vi "Signal Table Anal.vi"(6 "error in (no error)":errorcluster caption="error in", 10 "Signal Table":string[][](table) caption="S Table", 11 "Signal Tag":string[](array[string])) -> (0 "MxRight":string[](array[string]), 1 "Assigned":string[](array[string]), 2 "RR":i32[](array[numeric]), 3 "AR":i32[](array[numeric]), 4 "error out":errorcluster, 5 "Direction":bool[](array[boolean]))   [LabVIEW 2018]
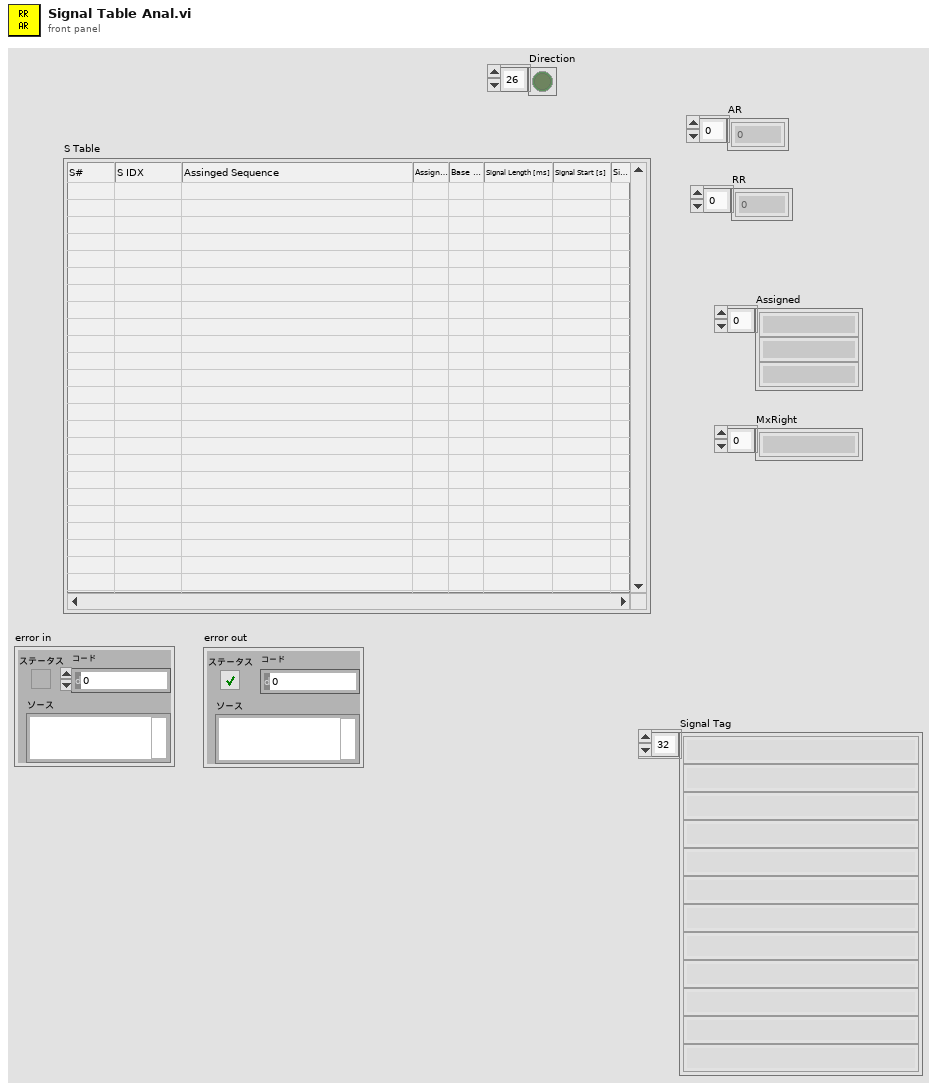
[diagram p1: front panel]
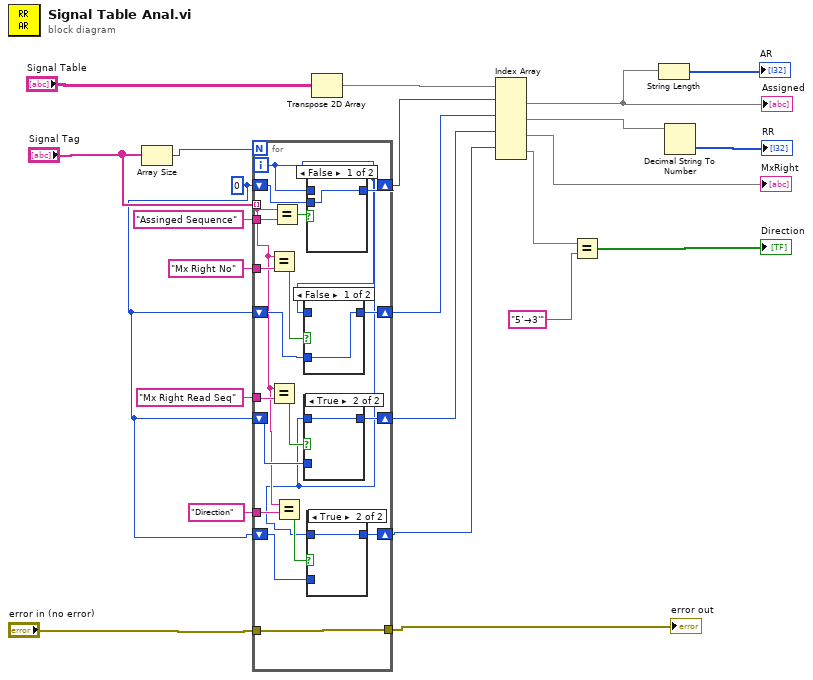
[diagram p0: block diagram]
diagram:
  w5 = 0
  n1 = Array Size(array="Signal Tag") -> (size(s)=w23:i32)
  n2 = for {
    N: w23 -> [_]
    tunnel: "Signal Tag" -> [w28] mode=indexing
    tunnel: "Assinged Sequence" ("グループ名入力") -> [w42]
    shift-right: [w40] -> w17
    shift-left: w5 -> [w41]
    tunnel: "Mx Right No" ("グループ名入力") -> [w36]
    shift-right: [w38] -> w16
    shift-left: w5 -> [w37]
    shift-right: [w32] -> w15
    shift-left: w5 -> [w31]
    tunnel: "Mx Right Read Seq" ("グループ名入力") -> [w33]
    tunnel: "error in (no error)" -> [w30]
    tunnel: [w30] -> w7
    tunnel: "Direction" ("グループ名入力") -> [w27]
    shift-right: [w25] -> w4
    shift-left: w5 -> [w26]
    i -> [w24]
    n3 = Equal?(x=w28, y=w36) -> (x = y?=w35:bool)
    n4 = Equal?(x=w28, y=w33) -> (x = y?=w34:bool)
    n5 = Equal?(x=w28, y=w42) -> (x = y?=w39:bool)
    n6 = Equal?(x=w28, y=w27) -> (x = y?=w29:bool)
    n7 = case shown="False" w35 {
      tunnel: w24 -> [_ w48]
      tunnel: [w47 w48] -> w38
      tunnel: w37 -> [w47 _]
      frame False {
      }
      frame True {
      }
    }
    n8 = case shown="True" w34 {
      tunnel: w24 -> [_ w46]
      tunnel: [w45 w46] -> w32
      tunnel: w31 -> [w45 _]
      frame False {
      }
      frame True {
      }
    }
    n9 = case shown="False" w39 {
      tunnel: w24 -> [_ w50]
      tunnel: [w49 w50] -> w40
      tunnel: w41 -> [w49 _]
      frame False {
      }
      frame True {
      }
    }
    n10 = case shown="True" w29 {
      tunnel: w24 -> [_ w44]
      tunnel: [w43 w44] -> w25
      tunnel: w26 -> [w43 _]
      frame False {
      }
      frame True {
      }
    }
  }
  "error out" <- w7
  n11 = Transpose 2D Array(2D array="Signal Table") -> (transposed array=w14:string[][])
  n12 = Index Array(array=w14, index (row) #1=w17, index (row) #2=w16, index (row) #3=w15, index (row) #4=w4) -> (element #1=w10:string[], element #2=w12:string[], element #3=→"MxRight":string[], element #4=w3:string[])  [unwired: 4 in]
  "Assigned" <- w10
  n13 = Equal?(x=w3, y="5’→3'" ("グループ名入力")) -> (x = y?=→"Direction":bool[])
  n14 = String Length(string=w10) -> (length=→"AR":i32[])
  n15 = Decimal String To Number(string=w12) -> (number=→"RR":i32[])  [unwired: 2 in, 1 out]
